vi "Webmessages.vi"() -> ()   [LabVIEW 2020]
uses:
  C:/Users/Simon/Documents/GitHub/LV-WebView2/Source/Libs/Microsoft.Web.WebView2.WinForms.dll
  Libs/Microsoft.Web.WebView2.WinForms.dll
  Webview2 Lib/WebView2 Control Object/Register Events.vi
  Webview2 Lib/WebView2 Control Object/Write Document Source.vi
  Webview2 Lib/WebView2 Control Object/WebView2 Control.lvclass
panel:
  in  "WebView2":refnum<k24>(container)
  in  "Background":u32(colorbox)
  in  "stop":bool
  in  "Set JS":bool
  in  "Msg":bool
  out "Message from Page":string
  in  "Message to Page":string
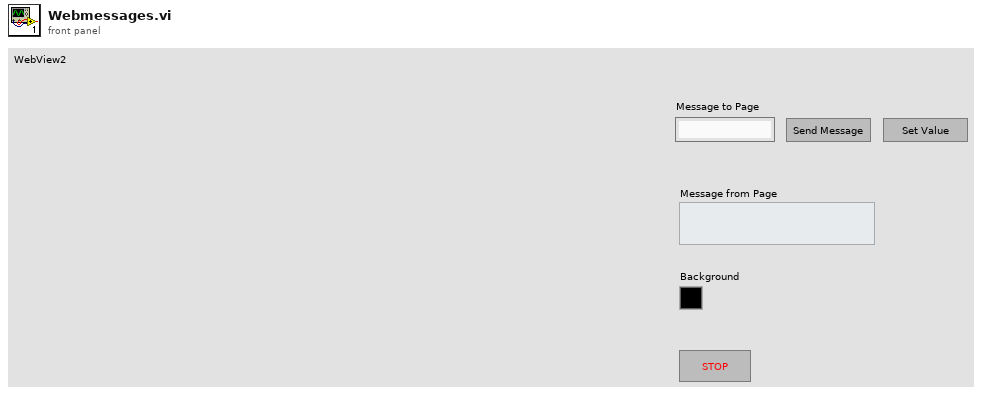
[diagram p1: front panel]
types:
  T1 = typedef "WebView2.lvlib/WebView2 Control.lvclass/Events.ctl" = cluster{"Navigation Complete Event":refnum<user-event>, "Source Changed Event":refnum<user-event>, "Document Title Changed Event":refnum<user-event>, "Status Bar Text Changed":refnum<user-event>, "Web Message Received":refnum<user-event>, "Window Close Requested":refnum<user-event>, "DOM Loaded":refnum<user-event>, "Navigation Started Event":refnum<user-event>}
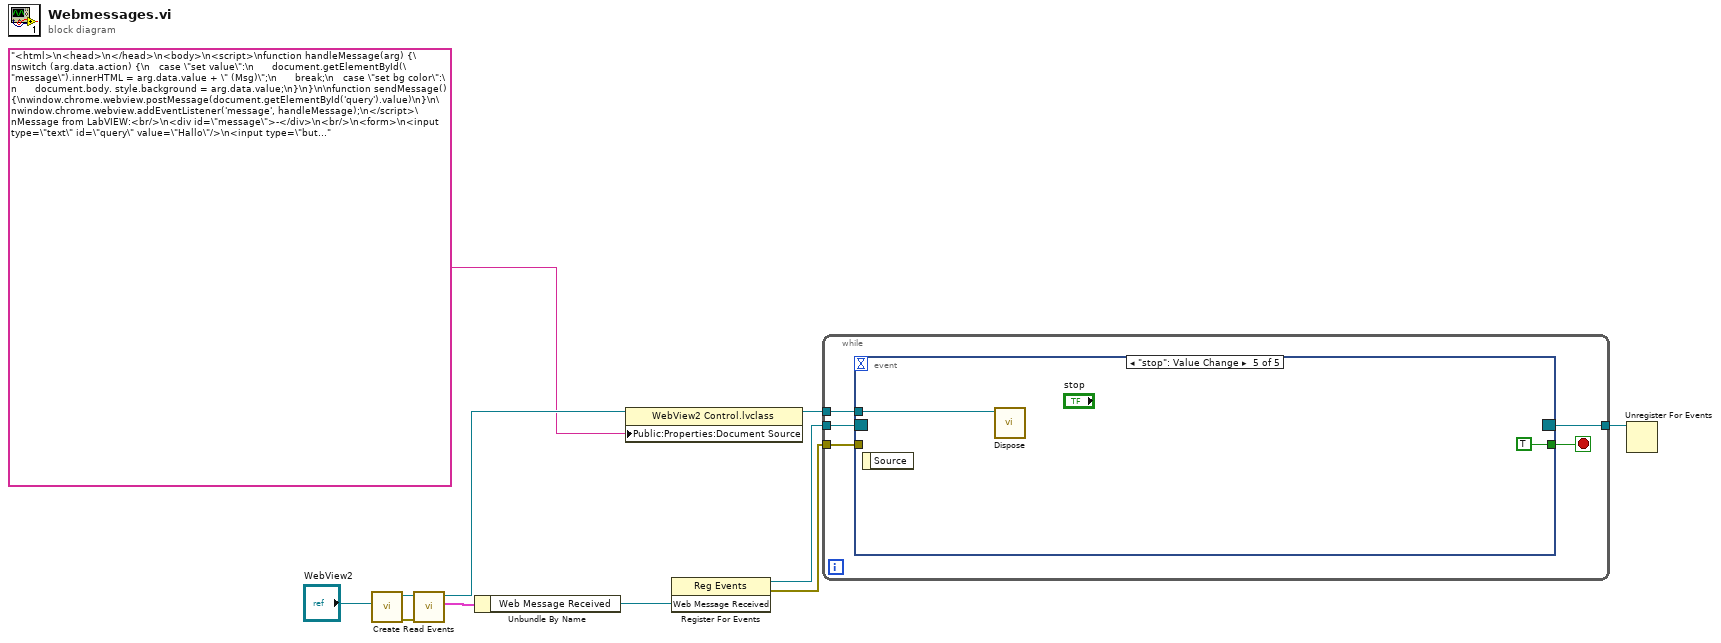
[diagram p0: block diagram]
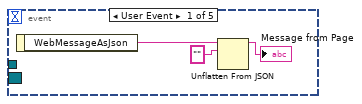
[diagram p2: hidden frame]
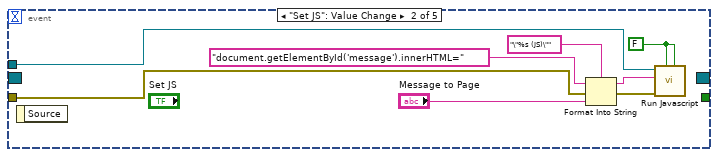
[diagram p3: hidden frame]
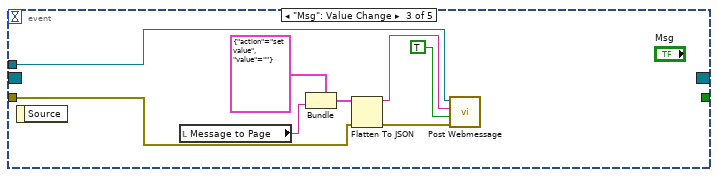
[diagram p4: hidden frame]
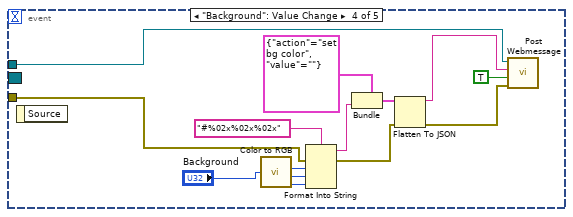
[diagram p5: hidden frame]
diagram:
  n1 = call "Create.vi"("WebView2 Control"="WebView2") -> ("error out"=w5:errorcluster, "WebView2 Control out"=w6:refnum<class "WebView2 Control.lvclass">)  [unwired: 9 in]
  n2 = call "Read Events.vi"("error in (no error)"=w5, "WebView2 Control in"=w6) -> ("Events"=w4:T1, "WebView2 Control out"=w3:refnum<class "WebView2 Control.lvclass">)  [unwired: 7 in, 1 out]
  n3 = Unbundle By Name(w4) -> ("Web Message Received"=w9:refnum<user-event>)
  n4 = property class="WebView2 Control.lvclass"(reference=w3, "Public:Properties:Document Source"="<html>\n<head>\n</head>\n<body>\n<script>\nfunction handleMessage(arg) {\nswitch (arg.data.action) {\n   case \"set value\":\n      document.getElementById(\"message\").innerHTML = arg.data.value + \" (Msg)\";\n      break;\n   case \"set bg color\":\n      document.body. style.background = arg.data.value;\n}\n}\n\nfunction sendMessage() {\nwindow.chrome.webview.postMessage(document.getElementById('query').value)\n}\n\nwindow.chrome.webview.addEventListener('message', handleMessage);\n</script>\nMessage from LabVIEW:<br/>\n<div id=\"message\">-</div>\n<br/>\n<form>\n<input type=\"text\" id=\"query\" value=\"Hallo\"/>\n<input type=\"button\" onclick=\"sendMessage()\" value=\"Send To LabVIEW\">\n</body>\n</html>" ("Document Source")) -> (reference out=w2:refnum<class "WebView2 Control.lvclass">)  [unwired: 1 in, 1 out]
  n5 = register-events(w9) -> (reference out=w11:refnum<event-registration>, error out=w10:errorcluster)  [unwired: 2 in]
  n6 = while {
    tunnel: w11 -> [w14]
    tunnel: w10 -> [w15]
    tunnel: [w13] -> w8
    tunnel: w2 -> [w12]
    stop <- w16 stop-if-true
    n7 = event shown="[4] \"stop\": Value Change" {
      selector: w14 -> [_ _ _ _ _]
      dyn-events: [_ _ _ _ _] -> w13
      timeout: _ -> [_ _ _ _ _]
      tunnel: [_ _ _ _ TRUE] -> w16
      tunnel: w15 -> [_ w24 w32 w40 _]
      tunnel: w12 -> [_ w23 w31 w39 w50]
      event User Event {
        n8 = event-data() -> ("WebMessageAsJson"=w19:string)  [unwired: 1 in]
        n9 = Unflatten From JSON(JSON string=w19, type and defaults="") -> (value=→"Message from Page":string)  [unwired: 5 in, 1 out]
      }
      event "Set JS": Value Change {
        w21 = FALSE ("Fetch Result")
        n10 = event-data() -> ()  [unwired: 1 in, 1 out]
        n11 = Format Into String(format string="\"%s (JS)\"", initial string="document.getElementById('message').innerHTML=" ("javaScript"), error in=w24, "Message to Page") -> (resulting string=w22:string, error out=w20:errorcluster)
        n12 = call "Run Javascript.vi"("Decode Result (T)"=w21, "Fetch Result (T)"=w21, "error in (no error)"=w20, "javaScript"=w22, "WebView2 Control in"=w23) -> ()  [unwired: 4 in, 3 out]
      }
      event "Msg": Value Change {
        n13 = event-data() -> ()  [unwired: 1 in, 1 out]
        n14 = local read "Message to Page"() -> (w33:string)
        n15 = Bundle(cluster=cluster{"action":string, "value":string} {"action"="set value", "value"=""}, "value"=w33) -> (w34:cluster{"action":string, "value":string})  [unwired: 1 in]
        n16 = Flatten To JSON(anything=w34, error in (no error)=w32) -> (JSON string=w29:string, 11:w28:errorcluster)  [unwired: 1 in]
        n17 = call "Post Webmessage.vi"("error in (no error)"=w28, "Send as JSON"=TRUE, "Message"=w29, "WebView2 Control in"=w31) -> ()  [unwired: 6 in, 2 out]
      }
      event "Background": Value Change {
        n18 = event-data() -> ()  [unwired: 1 in, 1 out]
        n19 = call <vilib>:"Color to RGB.vi"("Color"="Background") -> ("R"=w43:u8, "G"=w42:u8, "B"=w41:u8)  [unwired: 1 out]
        n20 = Format Into String(format string="#%02x%02x%02x", error in=w40, w43, w42, w41) -> (resulting string=w46:string, error out=w45:errorcluster)  [unwired: 1 in]
        n21 = Bundle(cluster=cluster{"action":string, "value":string} {"action"="set bg color", "value"=""}, "value"=w46) -> (w48:cluster{"action":string, "value":string})  [unwired: 1 in]
        n22 = Flatten To JSON(anything=w48, error in (no error)=w45) -> (JSON string=w38:string, 11:w37:errorcluster)  [unwired: 1 in]
        n23 = call "Post Webmessage.vi"("error in (no error)"=w37, "Send as JSON"=TRUE, "Message"=w38, "WebView2 Control in"=w39) -> ()  [unwired: 6 in, 2 out]
      }
      event "stop": Value Change {
        n24 = event-data() -> ()  [unwired: 1 in, 1 out]
        n25 = call "Dispose.vi"("WebView2 Control in"=w50) -> ()  [unwired: 10 in, 1 out]
      }
    }
  }
  n26 = Unregister For Events(event registration refnum=w8) -> ()  [unwired: 1 in, 1 out]
